vi "Dashboard Main.vi"() -> ()   [LabVIEW 2017]
uses:
  <vilib>/Rock Robotics/Network Tables/NT Read Numeric Array.vi
  <vilib>/Rock Robotics/Network Tables/NT Read Boolean.vi
  <vilib>/Rock Robotics/Network Tables/NT Read String.vi
  <vilib>/Rock Robotics/Network Tables/NT Read Number.vi
  <vilib>/Rock Robotics/WPI/Dashboard/WPI_DashboardLogging Global.vi
  <vilib>/Rock Robotics/Network Tables/NT Write Boolean.vi
  <vilib>/Rock Robotics/Network Tables/NT Read String Array.vi
  <vilib>/Rock Robotics/Network Tables/NT Write Number.vi
panel:
  in  "Camera Name":string(combo)="No Camera Selection"
  in  "Camera Settings Right":T1={"Frame Rate"=30, "Compression"=30, "Size"=1, "DB Camera Config"=FALSE} {"Frame Rate" scale=1.0..30.0; "Compression" scale=100.0..-1.0; "Size" items=["640x480", "320x240", "160x120"]}
  in  "Camera Name Right":string(combo)="No Camera Selection"
  out "Camera Info":cluster{"Mbps LED":bool, "Mbps":dbl, "fps":dbl} {"fps" format="%#.1g"; "Mbps" format="%#.1g"}
  in  "Camera Settings":T1={"Frame Rate"=30, "Compression"=30, "Size"=1, "DB Camera Config"=FALSE} {"Frame Rate" scale=1.0..30.0; "Compression" scale=100.0..-1.0; "Size" items=["640x480", "320x240", "160x120"]}
  in  "TCP":refnum<k5>
  in  "Rec Mode":enum32{"Stop", "Record", "Playback"}(radio)
  out "Robot IP":string
  out "Image Message":string="Timeout in Camera Communications"
  in  "Dashboard Tab":T2(tab)
  out "NT Connection":bool
  out "MotorChart R":cluster{"Numeric":dbl, "Numeric":dbl}(graph)
  out "MotorChart L":cluster{"Numeric":dbl, "Numeric":dbl}(graph)
  out "MotorSliders R":cluster{"MotorSlide1":dbl, "MotorSlide2":dbl} {"MotorSlide2" scale=-1.0..1.0 scale format="%#_2e"; "MotorSlide1" scale=-1.0..1.0 scale format="%#_2e"}
  out "MotorSliders L":cluster{"MotorSlide1":dbl, "MotorSlide2":dbl} {"MotorSlide2" scale=-1.0..1.0 scale format="%#_2e"; "MotorSlide1" scale=-1.0..1.0 scale format="%#_2e"}
  out "Gyro":dbl(knob) scale=0.0..360.0
  out "JS1 Z":dbl(slide) scale=-1.0..1.0 scale format="%#_2e"
  out "JS1 Graph":cluster{"X":dbl, "Y":dbl}[](graph)
  out "JS1 Buttons":T3
  out "JS2 Z":dbl(slide) scale=-1.0..1.0 scale format="%#_2e"
  out "JS2 Graph":cluster{"X":dbl, "Y":dbl}[](graph)
  out "JS2 Buttons":T3
  out "Mode":T4(ring)=enum."Auto Disabled"
  in  "Reload Auto Routines":bool
  in  "Starting Position":u16(ring) items=["Any", "Left", "Center", "Right"]
  in  "Run Auto In Teleop":bool
  in  "Right-Right-Right Routine":u16(ring) items=["Auto Line", "Auto Line (Reverse)", "Left Switch->Left Scale", "Left Switch->Left Switch->Left Scale", "Left Switch->Left Switch", "Left Switch->Left Switch (Back)", "Left Switch->Right Scale", "Left Switch", "Right Switch->Left Scale", "Right Switch->Right Scale", "Right Switch->Right Switch->Right Scale", "Right Switch->Right Switch", "Right Switch->Right Switch (Back)", "Right Switch"]
  in  "Right-Left-Right Routine":u16(ring) items=["Auto Line", "Auto Line (Reverse)", "Left Switch->Left Scale", "Left Switch->Left Switch->Left Scale", "Left Switch->Left Switch", "Left Switch->Left Switch (Back)", "Left Switch->Right Scale", "Left Switch", "Right Switch->Left Scale", "Right Switch->Right Scale", "Right Switch->Right Switch->Right Scale", "Right Switch->Right Switch", "Right Switch->Right Switch (Back)", "Right Switch"]
  in  "Left-Right-Left Routine":u16(ring) items=["Auto Line", "Auto Line (Reverse)", "Left Switch->Left Scale", "Left Switch->Left Switch->Left Scale", "Left Switch->Left Switch", "Left Switch->Left Switch (Back)", "Left Switch->Right Scale", "Left Switch", "Right Switch->Left Scale", "Right Switch->Right Scale", "Right Switch->Right Switch->Right Scale", "Right Switch->Right Switch", "Right Switch->Right Switch (Back)", "Right Switch"]
  in  "Left-Left-Left Routine":u16(ring) items=["Auto Line", "Auto Line (Reverse)", "Left Switch->Left Scale", "Left Switch->Left Switch->Left Scale", "Left Switch->Left Switch", "Left Switch->Left Switch (Back)", "Left Switch->Right Scale", "Left Switch", "Right Switch->Left Scale", "Right Switch->Right Scale", "Right Switch->Right Switch->Right Scale", "Right Switch->Right Switch", "Right Switch->Right Switch (Back)", "Right Switch"]
  out "RRR":string
  out "RLR":string
  out "LRL":string
  out "LLL":string
  out "Arm Control State":string
  out "Auto Control Active":bool
  out "Active Auto Routine":string
  out "Active Start Position":string
  out "Arm Rotate Limit Active":bool
  out "Arm Extend Limit Active":bool
  out "Arm Home Failure":bool
  out "Arm Home Success":bool
  out "Arm":cluster{dbl[], dbl[]}[](graph)
  out "Right Drive Zero":i32
  out "Left Drive Zero":i32
  in  "Reset Encoder Values":bool
  out "Right Drive":i32
  out "Left Drive":i32
  out "Tree":string(tree)
  out "Camera Image":T5(plugin-control)
  # "HW"
  # "HW"
  # "Joysticks"
  # "Drive Motors"
  # "Front"
  # "Right"
  # "Left"
  # "Back"
  # "Left Start"
  # "Center Start"
  # "Right Start"
  # "Armed Auto Routines"
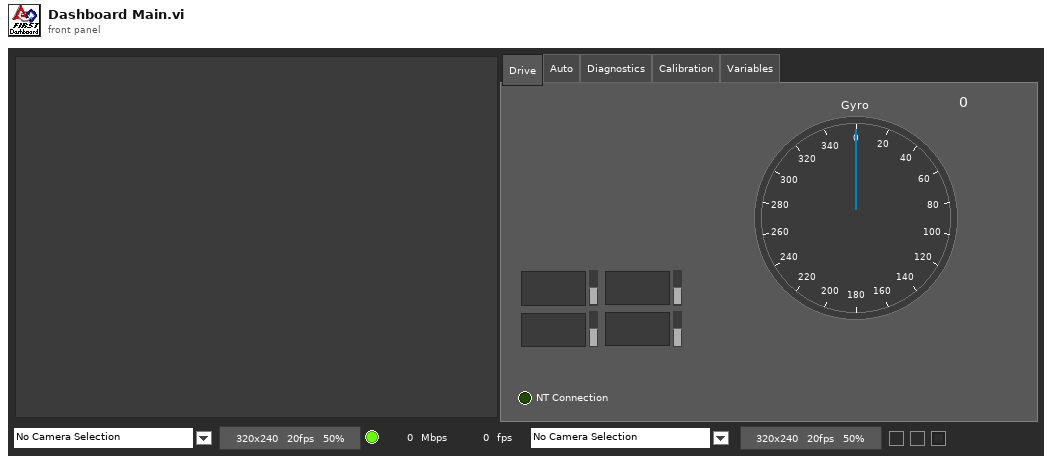
[diagram p1: front panel]
types:
  T1 = cluster{"Frame Rate":i32, "Compression":i32, "Size":u16, "DB Camera Config":bool}
  T2 = enum32{"Drive", "Auto", "Diagnostics", "Calibration", "Variables"}
  T3 = cluster{bool, bool, bool, bool, bool, bool, bool, bool, bool, bool, bool, bool}
  T4 = enum8{"Tele-Op Disabled", "Tele-Op Enabled", "Auto Disabled", "Auto Enabled", "Test Disabled", "Test Enabled", "Disconnected", "No Code", "E-Stop"}
  T5 = typedef "IMAQ Image.ctl" = refnum<image>
  T6 = enum32{"Drive", "Auto", "Diagnostics", "Variables"}
  T7 = cluster{"Save Path":path, "Interval (s)":dbl, "Keep":i32}
  T8 = typedef "Image Type" = u32
  T9 = cluster{"IDs":cluster{"RPC field ID":u16, "Unique ID":u16}, "String":string}
  T10 = cluster{"Error Strings":string, "Disable Counts":cluster{u16, u16}, "Rail Faults":cluster{u16, u16, u16}, "Robot IP":string, "DB Mode":u8, "Event Info":cluster{"Name":string, "Type":u8, "Number":u16, "Replay":u8}}
  T11 = cluster{"Storage":cluster{"Disk Free":u64, "RAM Block":u32, "RAM free":u32}, "CPU Utilization":cluster{"CPU % ISR":sgl, "CPU % Time Crit":sgl, "CPU % Timed Str":sgl, "CPU % High":sgl, "CPU % Above":sgl, "CPU % Normal":sgl, "CPU % Low":sgl}, "CAN":cluster{"% Bus Utilization":sgl, "Bus Off Cnt":u32, "TX_FIFO Full Cnt":u32, "Receive Error Cnt":u8, "Transmit Error Cnt":u8}, "HID":cluster{"HID Outputs":u32, "Rumble Low":u16, "Rumble High":u16}[]}
  T12 = cluster{"Status bits":cluster{"Test Mode":bool, "Autonomous":bool, "Enabled":bool, "Code Start":bool, "Brownout":bool, "Reserved 2":bool, "Reserved 3":bool, "E-Stop":bool}, "Code Trace":cluster{"Disabled":bool, "TeleOp":bool, "Auto":bool, "Test":bool}, "Controller Type":enum16{"unknown", "cRIO", "roboRio"}, "Code?":enum16{"unknown", "noCode", "code"}, "Battery V":dbl}
  T13 = cluster{"Control Bits":cluster{"TestMode":bool, "Autonomous":bool, "Enabled":bool, "FMS Present":bool, bool, bool, bool, "E-Stop":bool}, "Team Station ":u8, "Countdown":sgl, "Joystick Values":cluster{"Axes":dbl[], "Buttons":bool[], "POVs":i16[]}[]}
  T14 = cluster{"Axes":dbl[], "Buttons":bool[], "POVs":i16[]}[]
  T15 = cluster{"Axes":dbl[], "Buttons":bool[], "POVs":i16[]}
  T16 = cluster{"Buttons[0]":bool, "Buttons[1]":bool, "Buttons[2]":bool, "Buttons[3]":bool, "Buttons[4]":bool, "Buttons[5]":bool, "Buttons[6]":bool, "Buttons[7]":bool, "Buttons[8]":bool, "Buttons[9]":bool, "Buttons[10]":bool, "Buttons[11]":bool}
  T17 = cluster{"Camera Image":refnum<vi>, "Dashboard Tab":refnum<vi>, "Rec Mode":refnum<vi>, "Tree":refnum<vi>, "Camera Settings":refnum<vi>, "Camera Name":refnum<vi>, "Camera Info":refnum<vi>, "Camera Settings Right":refnum<vi>, "Camera Name Right":refnum<vi>}
  T18 = cluster{"Camera Name Right":string, string, "Saved DB Images Info":cluster{"Save Path":path, "Interval (s)":dbl, "Keep":i32}}
  T19 = cluster{"Camera Name":string, string, "Saved DB Images Info":cluster{"Save Path":path, "Interval (s)":dbl, "Keep":i32}}
  T20 = cluster{"Operation":enum16{"Update", "Clear"}, "Color Box":u32}[]
  T21 = cluster{"Image Size":bool, "Image Type":bool, "Pixel Value":bool, "ROI Information":bool, "Zoom Factor":bool}
  T22 = cluster{"Shift":bool, "Ctrl":bool, "Alt":bool, "Cmd":bool, "Opt":bool}
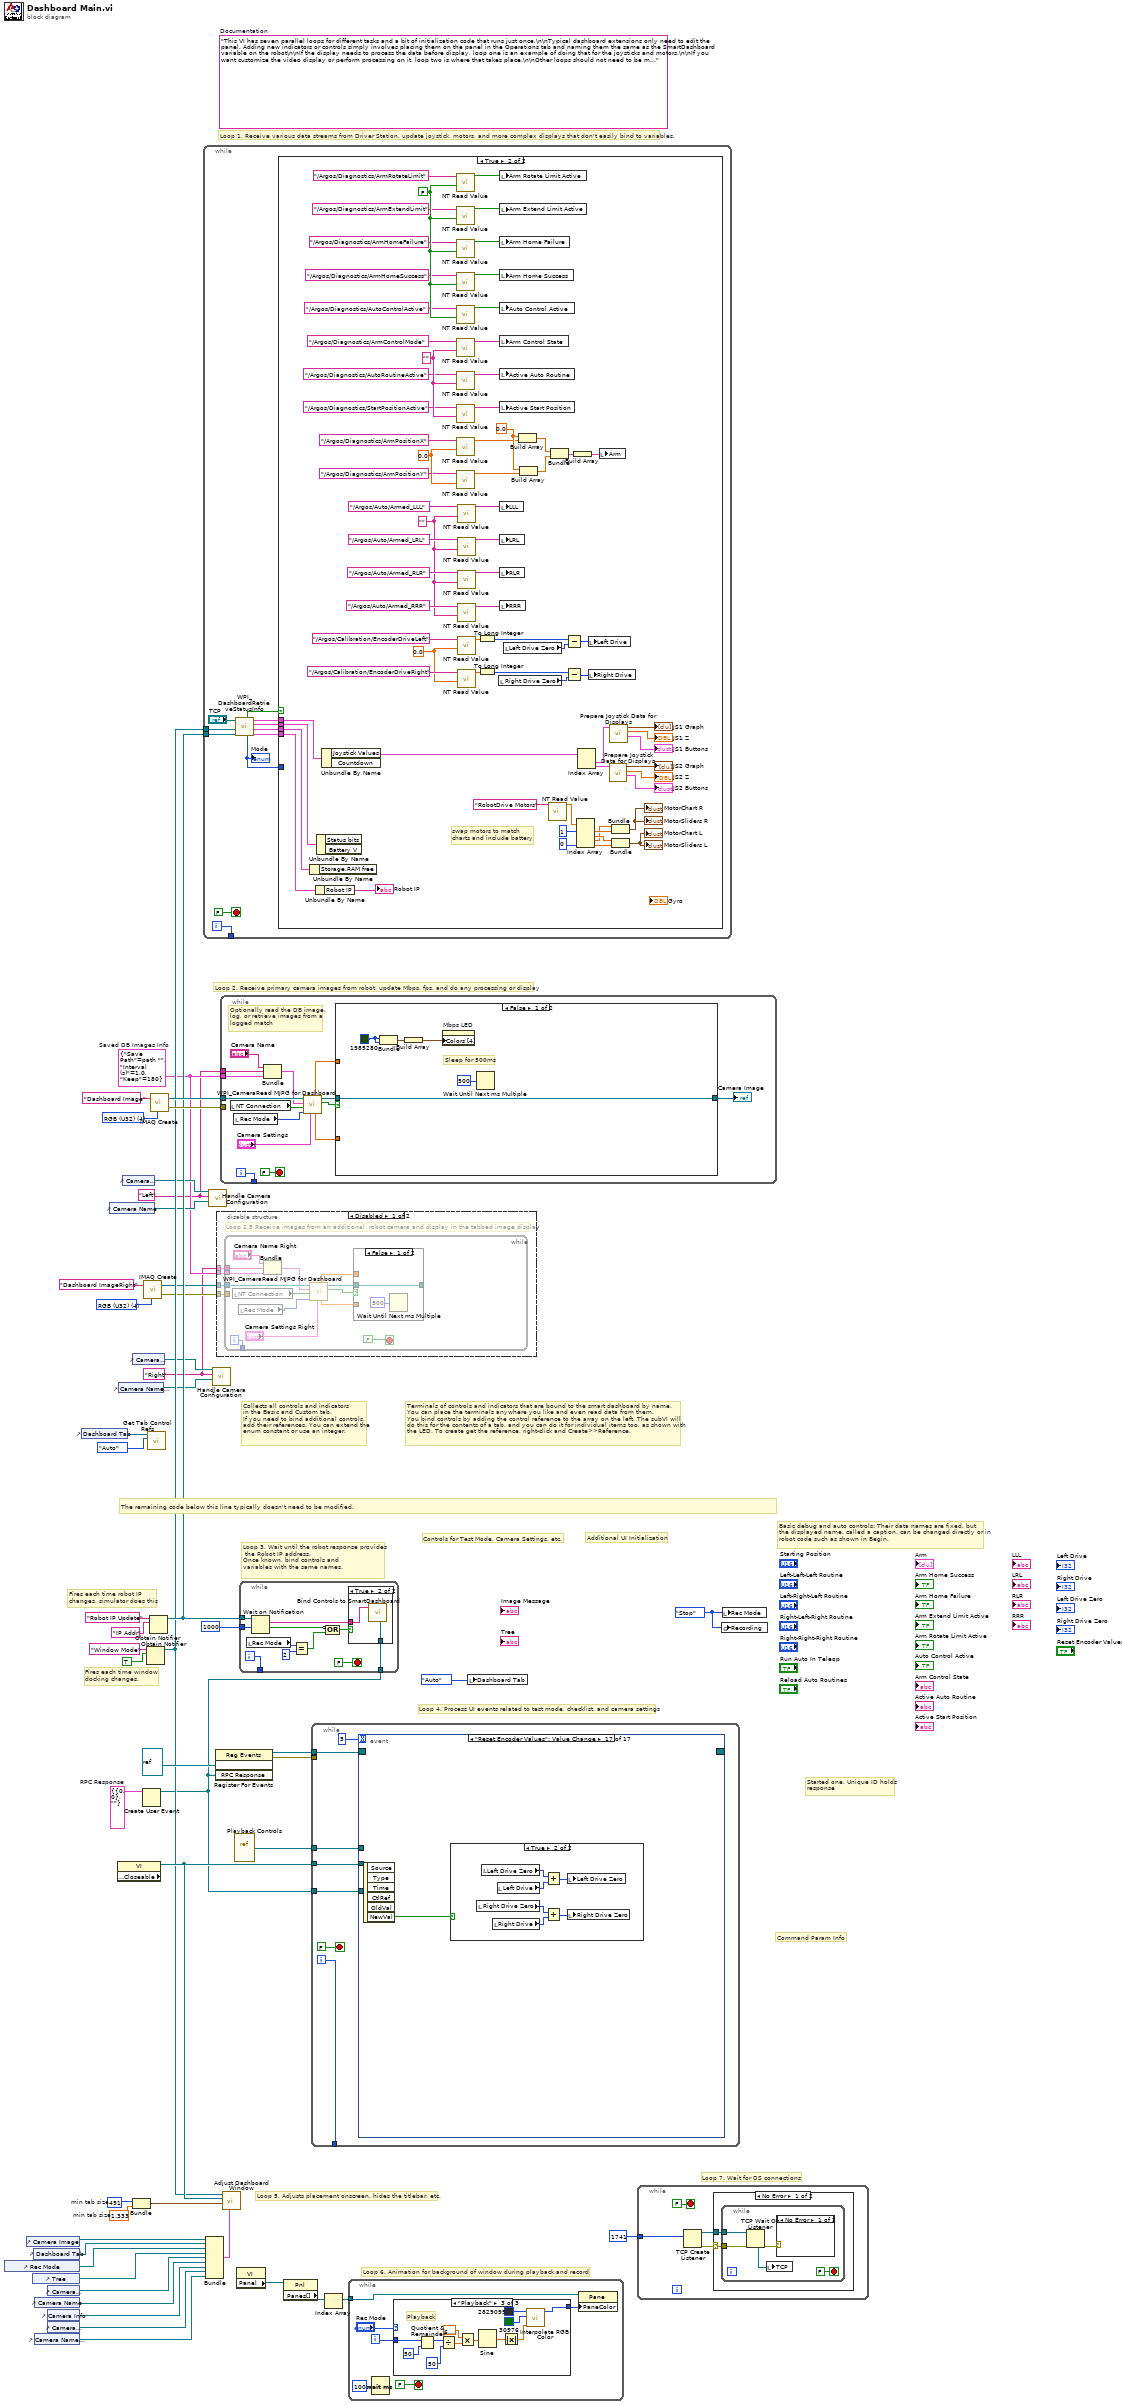
[diagram p0: block diagram]
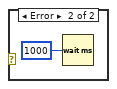
[diagram p5: hidden frame]
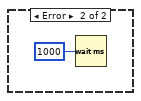
[diagram p6: hidden frame]
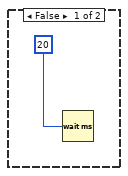
[diagram p7: hidden frame]
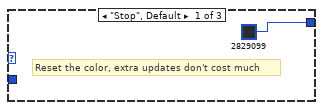
[diagram p8: hidden frame]
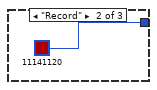
[diagram p9: hidden frame]
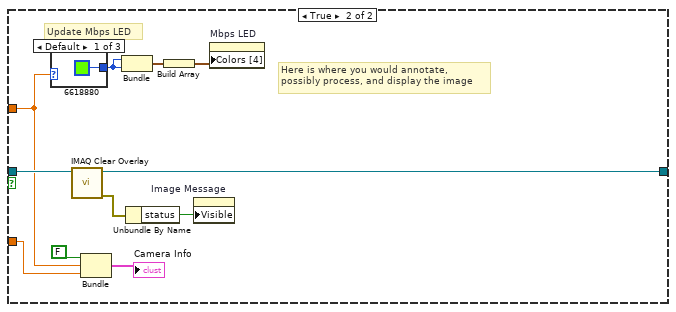
[diagram p10: hidden frame]
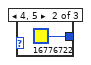
[diagram p11: hidden frame]
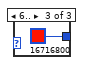
[diagram p12: hidden frame]
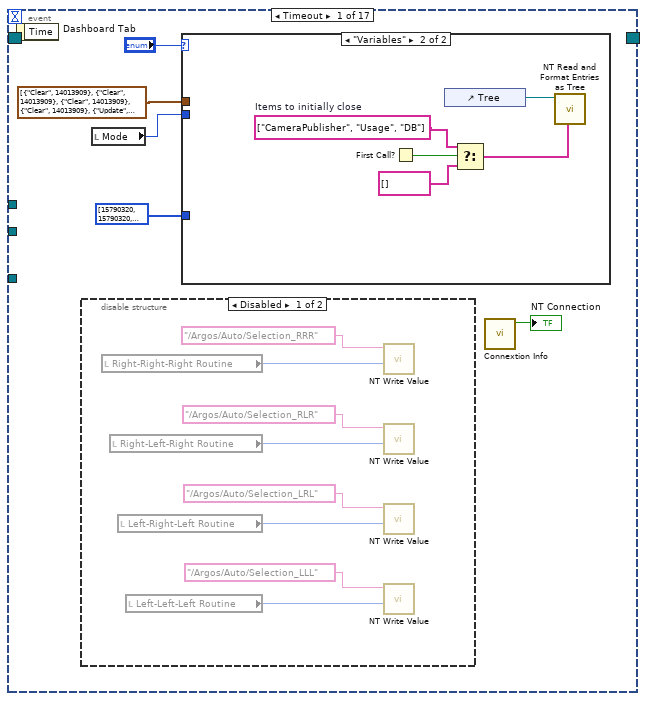
[diagram p13: hidden frame]
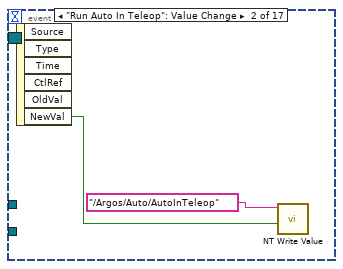
[diagram p16: hidden frame]
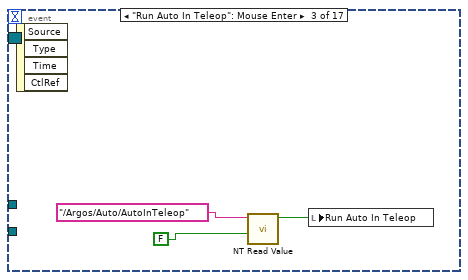
[diagram p17: hidden frame]
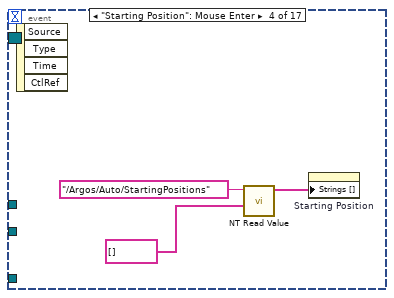
[diagram p18: hidden frame]
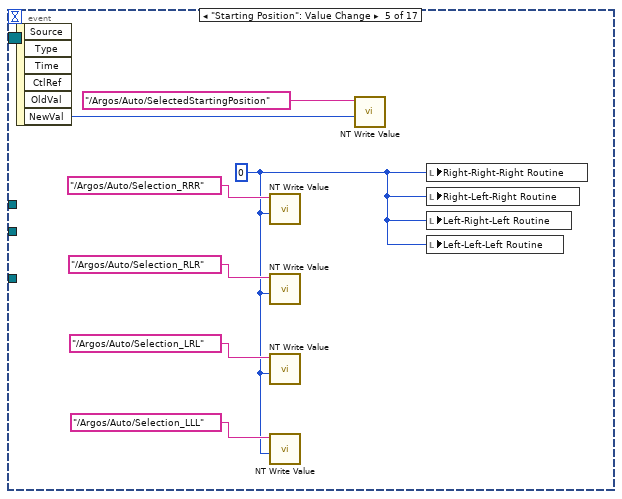
[diagram p19: hidden frame]
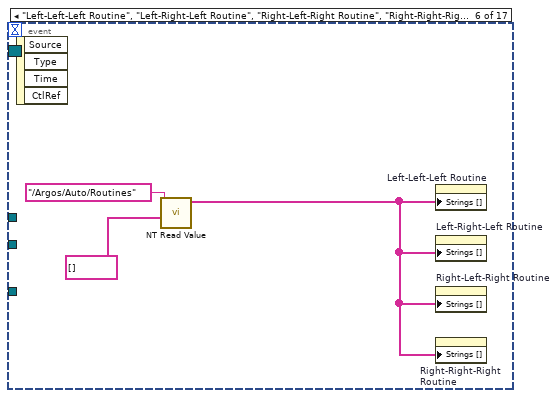
[diagram p20: hidden frame]
diagram:
  w5 = T7 {"Save Path"=path "", "Interval (s)"=1.0, "Keep"=180}  # Saved DB Images Info
  w4 = "Right"
  w3 = "Left"
  w12 = T8 4 items=["Grayscale (U8)", "Grayscale (I16)", "Grayscale (SGL)", "Complex (CSG)", "RGB (U32)", "HSL (U32)", "RGB (U64)"] ("Image Type")
  w20 = T9 {"IDs"={"RPC field ID"=0, "Unique ID"=0}, "String"=""}  # RPC Response
  w30 = 491  # min tab size
  w29 = 1.333  # min tab size
  w35 = enum32{"Stop", "Record", "Playback"}."Stop" ("Rec Mode")
  (unwired) "This VI has seven parallel loops for different tasks and a bit of initialization code that runs just once.\n\nTypical dashboard extensions only need to edit the panel. Adding new indicators or controls simply involves placing them on the panel in the Operations tab and naming them the same as the SmartDashboard variable on the robot\n\nIf the display needs to process the data before display, loop one is an example of doing that for the joysticks and motors.\n\nIf you want customize the video display or perform processing on it, loop two is where that takes place.\n\nOther loops should not need to be modified. They are pretty standard, and document the task they perform."  # Documentation
  w50 = T8 4 items=["Grayscale (U8)", "Grayscale (I16)", "Grayscale (SGL)", "Complex (CSG)", "RGB (U32)", "HSL (U32)", "RGB (U64)"] ("Image Type")
  # "Loop 3. Wait until the robot response provides\n the Robot IP address.\nOnce known, bind controls and\nvariables with the same names."
  # "Command Param Info"
  # "Started one, Unique ID holds\nresponse"
  # "Loop 7. Wait for DS connections"
  # "Basic debug and auto controls: Their data names are fixed, but\nthe displayed name, called a caption, can be changed directly or in\nrobot code such as shown in Begin."
  # "Controls for Test Mode, Camera Settings, etc."
  # "Additional UI Initialization"
  # "Loop 6. Animation for background of window during playback and record"
  # "Fires each time robot IP\nchanges, simulator does this"
  # "Fires each time window\ndocking changes."
  # "Collects all controls and indicators\nin the Basic and Custom tab.\nIf you need to bind additional controls,\nadd their references. You can extend the\nenum constant or use an integer."
  # "The remaining code below this line typically doesn't need to be modified."
  # "Loop 4. Process UI events related to test mode, checklist, and camera settings"
  # "Terminals of controls and indicators that are bound to the smart dashboard by name.\nYou can place the terminals anywhere you like and even read data from them.\nYou bind controls by adding the control reference to the array on the left. The subVI will\ndo this for the contents of a tab, and you can do it for individual items too, as shown with\nthe LED. To create get the reference, right-click and Create>>Reference."
  # "Loop 5. Adjusts placement onscreen, hides the titlebar, etc."
  # "Loop 1. Receive various data streams from Driver Station, update joystick, motors, and more complex displays that don't easily bind to variables."
  # "Loop 2. Receive primary camera images from robot, update Mbps, fps, and do any processing or display"
  n1 = control-ref of="Rec Mode"() -> (w25:refnum<vi>)
  n2 = control-ref of="Camera Image"() -> (w32:refnum<vi>)
  n3 = control-ref of="Tree"() -> (w26:refnum<vi>)
  n4 = control-ref of="Dashboard Tab"() -> (w31:refnum<vi>)
  n5 = control-ref of="Camera Name"() -> (w15:refnum<vi>)
  n6 = control-ref of="Camera Name Right"() -> (w6:refnum<vi>)
  n7 = control-ref of="Camera Settings"() -> (w16:refnum<vi>)
  n8 = control-ref of="Camera Info"() -> (w14:refnum<vi>)
  n9 = control-ref of="Camera Settings Right"() -> (w7:refnum<vi>)
  n10 = control-ref of="Dashboard Tab"() -> (w33:refnum<vi>)
  n11 = control-ref of="Camera Name"() -> (w17:refnum<vi>)
  n12 = property class="VI" props=["Front Panel.Closeable"]() -> (reference out=w34:refnum<vi>)  [unwired: 2 in, 2 out]
  n13 = control-ref of="Camera Name Right"() -> (w8:refnum<vi>)
  n14 = control-ref of="Camera Settings"() -> (w18:refnum<vi>)
  n15 = control-ref of="Camera Settings Right"() -> (w9:refnum<vi>)
  n16 = Bundle("min tab size"=w30, "min tab size"=w29) -> (w28:cluster{"min tab size":i32, "min tab size":dbl})  [unwired: 1 in]
  n17 = Create User Event(user event datatype=w20) -> (user event=w19:refnum<user-event>)  [unwired: 1 in, 1 out]
  n18 = call "IMAQ Create"("Image Name"="Dashboard ImageRight", "Image Type"=w12) -> ("New Image"=w11:T5, "error out"=w10:errorcluster)  [unwired: 2 in, 1 out]
  n19 = Obtain Notifier(name (unnamed)="Window Mode", notification data type=TRUE) -> (notifier out=w23:refnum<notifier>)  [unwired: 2 in, 2 out]
  n20 = call <vilib>:"Get Tab Control Refs.vi"("Page Index"=T6."Auto" ("Dashboard Tab"), "TabControl in"=w33) -> ()  [unwired: 9 in, 1 out]
  n21 = Obtain Notifier(name (unnamed)="Robot IP Update", notification data type="IP Addr" ("name (unnamed)")) -> (notifier out=w24:refnum<notifier>)  [unwired: 2 in, 2 out]
  n22 = call "IMAQ Create"("Image Name"="Dashboard Image", "Image Type"=w50) -> ("New Image"=w48:T5, "error out"=w47:errorcluster)  [unwired: 2 in, 1 out]
  n23 = while {
    tunnel: [w60] -> _
    tunnel: w24 -> [w54]
    tunnel: w23 -> [w51]
    i -> [w60]
    stop <- FALSE stop-if-true
    n24 = call <vilib>:"WPI_DashboardRetrieveStatusInfo.vi"("Binding Refnum"=w54, "Window Mode Notifier"=w51, "TCP Cnx"="TCP") -> ("Power and Errors"=w55:T10, "Robot Metrics"=w58:T11, "Status Info"=w59:T12, "Control Info"=w56:T13, "Robot Mode"=w53:T4, "Process?"=w57:bool)  [unwired: 3 in]
    "Mode" <- w53
    n25 = case shown="True" w57 {
      tunnel: w59 -> [_ w134]
      tunnel: w58 -> [_ w133]
      tunnel: w56 -> [_ w132]
      tunnel: w55 -> [_ w131]
      tunnel: w53 -> [_ _]
      frame False {
        n26 = Wait (ms)(milliseconds to wait=u32 20) -> ()  [unwired: 1 out]
      }
      frame True {
        w71 = 0.0 ("Default Value")
        w78 = "" ("Default Value")
        w88 = 0.0 ("Default Value")
        w93 = 0.0 ("element")
        w99 = "" ("Default Value")
        w110 = FALSE ("Default Value")
        # "swap motors to match\ncharts and include battery"
        n27 = Unbundle By Name(w133) -> ()  [unwired: 1 out]
        n28 = Unbundle By Name(w131) -> ("Robot IP"=→"Robot IP":string)
        n29 = Unbundle By Name(w134) -> ()  [unwired: 2 out]
        n30 = Unbundle By Name(w132) -> ("Joystick Values"=w122:T14)  [unwired: 1 out]
        n31 = call-poly <vilib>:"NT Read Value.vi"("Default Value"=w110, "Name"="/Argos/Diagnostics/ArmRotateLimit") -> ("Boolean"=w109:bool)  [unwired: 8 in, 1 out]
        n32 = call-poly <vilib>:"NT Read Value.vi"("Default Value"=w110, "Name"="/Argos/Diagnostics/ArmExtendLimit") -> ("Boolean"=w108:bool)  [unwired: 8 in, 1 out]
        n33 = call-poly <vilib>:"NT Read Value.vi"("Default Value"=w110, "Name"="/Argos/Diagnostics/ArmHomeFailure") -> ("Boolean"=w107:bool)  [unwired: 8 in, 1 out]
        n34 = call-poly <vilib>:"NT Read Value.vi"("Default Value"=w110, "Name"="/Argos/Diagnostics/ArmHomeSuccess") -> ("Boolean"=w106:bool)  [unwired: 8 in, 1 out]
        n35 = call-poly <vilib>:"NT Read Value.vi"("Default Value"=w110, "Name"="/Argos/Diagnostics/AutoControlActive") -> ("Boolean"=w105:bool)  [unwired: 8 in, 1 out]
        n36 = call-poly <vilib>:"NT Read Value.vi"("Default Value"=w99, "Name"="/Argos/Diagnostics/ArmControlMode") -> ("String"=w98:string)  [unwired: 8 in, 1 out]
        n37 = call-poly <vilib>:"NT Read Value.vi"("Default Value"=w99, "Name"="/Argos/Diagnostics/AutoRoutineActive") -> ("String"=w97:string)  [unwired: 8 in, 1 out]
        n38 = call-poly <vilib>:"NT Read Value.vi"("Default Value"=w99, "Name"="/Argos/Diagnostics/StartPositionActive") -> ("String"=w96:string)  [unwired: 8 in, 1 out]
        n39 = call-poly <vilib>:"NT Read Value.vi"("Default Value"=w88, "Name"="/Argos/Diagnostics/ArmPositionX") -> ("Numeric"=w92:dbl)  [unwired: 8 in, 1 out]
        n40 = call-poly <vilib>:"NT Read Value.vi"("Default Value"=w88, "Name"="/Argos/Diagnostics/ArmPositionY") -> ("Numeric"=w91:dbl)  [unwired: 8 in, 1 out]
        n41 = call-poly <vilib>:"NT Read Value.vi"("Default Value"=w78, "Name"="/Argos/Auto/Armed_LLL") -> ("String"=w77:string)  [unwired: 8 in, 1 out]
        n42 = call-poly <vilib>:"NT Read Value.vi"("Default Value"=w78, "Name"="/Argos/Auto/Armed_LRL") -> ("String"=w76:string)  [unwired: 8 in, 1 out]
        n43 = call-poly <vilib>:"NT Read Value.vi"("Default Value"=w78, "Name"="/Argos/Auto/Armed_RLR") -> ("String"=w75:string)  [unwired: 8 in, 1 out]
        n44 = call-poly <vilib>:"NT Read Value.vi"("Default Value"=w78, "Name"="/Argos/Auto/Armed_RRR") -> ("String"=w74:string)  [unwired: 8 in, 1 out]
        n45 = call-poly <vilib>:"NT Read Value.vi"("Default Value"=w71, "Name"="/Argos/Calibration/EncoderDriveLeft") -> ("Numeric"=w70:dbl)  [unwired: 8 in, 1 out]
        n46 = call-poly <vilib>:"NT Read Value.vi"("Default Value"=w71, "Name"="/Argos/Calibration/EncoderDriveRight") -> ("Numeric"=w69:dbl)  [unwired: 8 in, 1 out]
        n47 = To Long Integer(number=w70) -> (32bit integer=w64:i32)
        n48 = To Long Integer(number=w69) -> (32bit integer=w67:i32)
        n49 = local read "Right Drive Zero"() -> (w66:i32)
        n50 = local write "Arm Rotate Limit Active"(w109) -> ()
        n51 = local write "Arm Extend Limit Active"(w108) -> ()
        n52 = local write "Arm Home Failure"(w107) -> ()
        n53 = local write "Arm Home Success"(w106) -> ()
        n54 = local write "Auto Control Active"(w105) -> ()
        n55 = local write "Arm Control State"(w98) -> ()
        n56 = local write "Active Auto Routine"(w97) -> ()
        n57 = local write "Active Start Position"(w96) -> ()
        n58 = local write "LLL"(w77) -> ()
        n59 = local write "LRL"(w76) -> ()
        n60 = local write "RLR"(w75) -> ()
        n61 = local write "RRR"(w74) -> ()
        n62 = local read "Left Drive Zero"() -> (w63:i32)
        n63 = Build Array(w93, w92) -> (w95:dbl[])
        n64 = Build Array(w93, w91) -> (w94:dbl[])
        n65 = call-poly <vilib>:"NT Read Value.vi"("Name"="RobotDrive Motors") -> ("Numeric Array"=w112:dbl[])  [unwired: 9 in, 1 out]
        n66 = Bundle(w95, w94) -> (w90:cluster{dbl[], dbl[]})  [unwired: 1 in]
        n67 = Subtract(x=w64, y=w63) -> (x-y=w65:i32)
        n68 = Subtract(x=w67, y=w66) -> (x-y=w68:i32)
        n69 = Build Array(w90) -> (w89:cluster{dbl[], dbl[]}[])
        n70 = Index Array(array=w112, index #1=1, index #4=0) -> (element #1=w126:dbl, element #2=w127:dbl, element #3=w125:dbl, element #4=w130:dbl)  [unwired: 2 in]
        n71 = Index Array(array=w122) -> (element #1=w121:T15, element #2=w117:T15)  [unwired: 2 in]
        n72 = local write "Left Drive"(w65) -> ()
        n73 = local write "Right Drive"(w68) -> ()
        n74 = local write "Arm"(w89) -> ()
        n75 = call "Prepare Joystick Data for Displays.vi"("Joystick Values"=w117) -> ("Buttons"=→"JS2 Buttons":T16, "Z Axis"=→"JS2 Z":dbl, "Cartesian Data"=→"JS2 Graph":cluster{"X axis":dbl, "X axis":dbl}[])  [unwired: 8 in]
        n76 = call "Prepare Joystick Data for Displays.vi"("Joystick Values"=w121) -> ("Buttons"=→"JS1 Buttons":T16, "Z Axis"=→"JS1 Z":dbl, "Cartesian Data"=→"JS1 Graph":cluster{"X axis":dbl, "X axis":dbl}[])  [unwired: 8 in]
        n77 = Bundle("Numeric"=w125, "Numeric"=w126) -> (→"MotorChart R" →"MotorSliders R":cluster{"Numeric":dbl, "Numeric":dbl})  [unwired: 1 in]
        n78 = Bundle("Numeric"=w127, "Numeric"=w130) -> (→"MotorChart L" →"MotorSliders L":cluster{"Numeric":dbl, "Numeric":dbl})  [unwired: 1 in]
      }
    }
  }
  n79 = Bundle("Camera Image"=w32, "Dashboard Tab"=w31, "Rec Mode"=w25, "Tree"=w26, "Camera Settings"=w16, "Camera Name"=w15, "Camera Info"=w14, "Camera Settings Right"=w7, "Camera Name Right"=w6) -> (w27:T17)  [unwired: 1 in]
  n80 = call "Handle Camera Configuration.vi"("CameraNameRef"=w17, "Display Name"=w3, "ClusterRef"=w18) -> ()  [unwired: 9 in]
  n81 = call "Handle Camera Configuration.vi"("CameraNameRef"=w8, "Display Name"=w4, "ClusterRef"=w9) -> ()  [unwired: 9 in]
  n82 = register-events(refnum<vi> refnum, w19) -> (reference out=w38:refnum<event-registration>, error out=w37:errorcluster)  [unwired: 2 in]
  n83 = disable-structure shown="Disabled" {
    disable-tunnel: w11 -> [w138 _]
    disable-tunnel: w10 -> [w137 _]
    disable-tunnel: w5 -> [w136 _]
    disable-tunnel: w4 -> [w135 _]
    frame Disabled {
      # "Loop 2.5 Receive images from an additional  robot camera and display in the tabbed image display"
      n84 = while {
        tunnel: w138 -> [w152]
        tunnel: w137 -> [_]
        tunnel: [w147] -> _
        tunnel: w136 -> [w142]
        tunnel: w135 -> [w139]
        i -> [w147]
        stop <- FALSE stop-if-true
        n85 = local read "NT Connection"() -> (w143:bool)
        n86 = local read "Rec Mode"() -> (w151:enum32{"Stop", "Record", "Playback"})
        n87 = Bundle("Camera Name Right"="Camera Name Right", w139, "Saved DB Images Info"=w142) -> (w141:T18)  [unwired: 1 in]
        n88 = call <vilib>:"WPI_CameraRead MJPG for Dashboard.vi"("Camera Settings"="Camera Settings Right", "Rec Mode"=w151, "NT Connection"=w143, "Capture Info"=w141, "Refnum in"=w152) -> ("Active"=w146:bool, "Refnum out"=w149:T5, "FPS"=w144:dbl, "Bandwidth (Mbps)"=w145:dbl)  [unwired: 3 in]
        n89 = case shown="False" w146 {
          tunnel: w149 -> [w153 w155]
          tunnel: w145 -> [_ _]
          tunnel: w144 -> [_ _]
          tunnel: [w153 w155] -> _
          frame False {
            n90 = Wait Until Next ms Multiple(millisecond multiple=u32 500) -> ()  [unwired: 1 out]
          }
          frame True {
          }
        }
      }
    }
    frame Enabled {
    }
  }
  n91 = while {
    tunnel: w48 -> [w168]
    tunnel: w47 -> [_]
    tunnel: [w169] -> _
    tunnel: w5 -> [w159]
    tunnel: w3 -> [w156]
    i -> [w169]
    stop <- FALSE stop-if-true
    # "Optionally read the DB image,\nlog, or retrieve images from a\nlogged match"
    n92 = local read "NT Connection"() -> (w160:bool)
    n93 = local read "Rec Mode"() -> (w164:enum32{"Stop", "Record", "Playback"})
    n94 = Bundle("Camera Name"="Camera Name", w156, "Saved DB Images Info"=w159) -> (w158:T19)  [unwired: 1 in]
    n95 = call <vilib>:"WPI_CameraRead MJPG for Dashboard.vi"("Camera Settings"="Camera Settings", "Rec Mode"=w164, "NT Connection"=w160, "Capture Info"=w158, "Refnum in"=w168) -> ("Active"=w166:bool, "Refnum out"=w167:T5, "FPS"=w165:dbl, "Bandwidth (Mbps)"=w163:dbl)  [unwired: 3 in]
    n96 = case shown="False" w166 {
      tunnel: w167 -> [w171 w182]
      tunnel: w163 -> [_ w179]
      tunnel: w165 -> [_ w180]
      tunnel: [w171 w176] -> w161
      frame False {
        w173 = u32 1985280 ("Color Box")
        # "Sleep for 500ms"
        n97 = Bundle("Color Box"=w173, "Color Box"=w173) -> (w174:cluster{"Color Box":u32, "Color Box":u32})  [unwired: 1 out]
        n98 = Build Array(w174) -> (w172:cluster{"Color Box":u32, "Color Box":u32}[])
        n99 = property on="Mbps LED" class="Bool (strict)"("Colors [4]"=w172) -> ()  [unwired: 2 in, 2 out]
        n100 = Wait Until Next ms Multiple(millisecond multiple=u32 500) -> ()  [unwired: 1 out]
      }
      frame True {
        # "Here is where you would annotate,\npossibly process, and display the image"
        # "Update Mbps LED"
        n101 = case shown="Default" w179 {
          tunnel: [u32 6618880 ("Color Box") u32 16776722 ("Color Box") u32 16716800 ("Color Box")] -> w183
          frame Default {
          }
          frame 4, 5 {
          }
          frame 6.. {
          }
        }
        n102 = call "IMAQ Clear Overlay"("Image"=w182) -> ("error out"=w185:errorcluster, "Image Out"=w176:T5)  [unwired: 2 in, 7 out]
        n103 = Bundle(FALSE, "Bandwidth (Mbps)"=w179, "FPS"=w180) -> (→"Camera Info":cluster{bool, "Bandwidth (Mbps)":dbl, "FPS":dbl})  [unwired: 1 in]
        n104 = Bundle("Color Box"=w183, "Color Box"=w183) -> (w184:cluster{"Color Box":u32, "Color Box":u32})  [unwired: 1 out]
        n105 = Unbundle By Name(w185) -> ("status"=w186:bool)
        n106 = Build Array(w184) -> (w181:cluster{"Color Box":u32, "Color Box":u32}[])
        n107 = property on="Image Message" class="Str"("Visible"=w186) -> ()  [unwired: 2 in, 2 out]
        n108 = property on="Mbps LED" class="Bool (strict)"("Colors [4]"=w181) -> ()  [unwired: 2 in, 2 out]
      }
    }
    "Camera Image" <- w161
  }
  n109 = call "Adjust Dashboard Window.vi"("Sizing Refnums"=w27, "Size Constraints"=w28, "VI"=w34, "WIn Mode"=w23) -> ()  [unwired: 8 in]
  n110 = vi-ref "Playback Controls.vi"() -> (w39:refnum<vi>)
  n111 = property class="VI"() -> ("Panel"=w41:refnum<vi>)  [unwired: 2 in, 2 out]
  n112 = while {
    tunnel: w24 -> [w199]
    tunnel: [w197] -> _
    tunnel: u32 1000 ("milliseconds to wait") -> [w196]
    tunnel: w19 -> [w190]
    i -> [w197]
    stop <- FALSE stop-if-true
    n113 = local read "Rec Mode"() -> (w192:enum32{"Stop", "Record", "Playback"})
    n114 = Wait on Notification(notifier=w199, timeout in ms (-1)=w196) -> (notification=w198:string, timed out?=w194:bool)  [unwired: 2 in, 2 out]
    n115 = Equal?(x=w192, y=u16 2 ("Rec Mode")) -> (x = y?=w193:bool)
    n116 = Compound Arithmetic op=OR(invert w194, w193) -> (w195:bool)
    n117 = case shown="True" w195 {
      tunnel: w198 -> [_ w202]
      tunnel: w190 -> [_ w201]
      frame False {
      }
      frame True {
        n118 = call <vilib>:"Bind Controls to SmartDashboard.vi"("RPC ref"=w201, "Server IP Address"=w202) -> ()  [unwired: 10 in]
      }
    }
  }
  n119 = property class="Pnl"(reference=w41) -> ("Panes[]"=w42:refnum<vi>[])  [unwired: 1 in, 2 out]
  n120 = while {
    tunnel: [w207] -> _
    tunnel: w39 -> [w206]
    tunnel: w38 -> [w205]
    tunnel: w37 -> [_]
    tunnel: w34 -> [w204]
    tunnel: w19 -> [w203]
    i -> [w207]
    stop <- FALSE stop-if-true
    n121 = event shown="[16] \"Reset Encoder Values\": Value Change" {
      selector: w205 -> [_ _ _ _ _ _ _ _ _ _ _ _ _ _ _ _ _]
      dyn-events: [_ _ _ _ _ _ _ _ _ _ _ _ w265 _ _ _ _] -> _
      timeout: u32 5 ("milliseconds to wait") -> [_ _ _ _ _ _ _ _ _ _ _ _ _ _ _ _ _]
      tunnel: w206 -> [_ _ _ _ _ _ _ _ _ _ _ _ w267 _ w283 _ _]
      tunnel: w204 -> [_ _ _ _ _ _ _ _ _ _ _ _ w263 _ _ _ _]
      tunnel: w203 -> [_ _ _ _ _ _ _ _ _ _ _ _ w261 _ _ _ _]
      event Timeout {
        n122 = event-data() -> ()  [unwired: 1 in, 1 out]
        n123 = disable-structure shown="Disabled" {
          frame Disabled {
            n124 = local read "Right-Right-Right Routine"() -> (w219:u16)
            n125 = local read "Right-Left-Right Routine"() -> (w220:u16)
            n126 = local read "Left-Right-Left Routine"() -> (w222:u16)
            n127 = local read "Left-Left-Left Routine"() -> (w221:u16)
            n128 = call-poly <vilib>:"NT Write Value.vi"("Numeric"=w219, "Name"="/Argos/Auto/Selection_RRR") -> ()  [unwired: 9 in, 1 out]
            n129 = call-poly <vilib>:"NT Write Value.vi"("Numeric"=w220, "Name"="/Argos/Auto/Selection_RLR") -> ()  [unwired: 9 in, 1 out]
            n130 = call-poly <vilib>:"NT Write Value.vi"("Numeric"=w222, "Name"="/Argos/Auto/Selection_LRL") -> ()  [unwired: 9 in, 1 out]
            n131 = call-poly <vilib>:"NT Write Value.vi"("Numeric"=w221, "Name"="/Argos/Auto/Selection_LLL") -> ()  [unwired: 9 in, 1 out]
          }
          frame Enabled {
          }
        }
        n132 = local read "Mode"() -> (w211:T4)
        n133 = case shown="\"Variables\"" "Dashboard Tab" {
          tunnel: T20 [{"Operation"=enum."Clear", "Color Box"=14013909}, {"Operation"=enum."Clear", "Color Box"=14013909}, {"Operation"=enum."Clear", "Color Box"=14013909}, {"Operation"=enum."Clear", "Color Box"=14013909}, {"Operation"=enum."Update", "Color Box"=14013909}, {"Operation"=enum."Update", "Color Box"=16777215}, {"Operation"=enum."Clear", "Color Box"=14013909}, {"Operation"=enum."Clear", "Color Box"=14013909}, {"Operation"=enum."Clear", "Color Box"=14013909}] -> [_ _]
          tunnel: w211 -> [_ _]
          tunnel: u32[] [15790320, 15790320, 15790320, 15790320, 16777215, 16777215, 15790320, 15790320, 15790320] -> [_ _]
          frame "Diagnostics", Default {
          }
          frame "Variables" {
            w225 = string[] ["CameraPublisher", "Usage", "DB"]  # Items to initially close
            n134 = First Call?() -> (First Call?: T/F=w226:bool)
            n135 = control-ref of="Tree"() -> (w227:refnum<vi>)
            n136 = Select(t=w225, s=w226, f=string[] []) -> (s? t:f=w223:string[])
            n137 = call <vilib>:"NT Read and Format Entries as Tree.vi"("Tags to  Close"=w223, "Tree Refnum"=w227) -> ()  [unwired: 8 in, 2 out]
          }
        }
        n138 = call <vilib>:"Connextion Info.vi"() -> ("Connected"=→"NT Connection":bool)  [unwired: 10 in, 1 out]
      }
      event "Run Auto In Teleop": Value Change {
        n139 = event-data() -> ("NewVal"=w229:bool)  [unwired: 1 in, 5 out]
        n140 = call-poly <vilib>:"NT Write Value.vi"("Boolean"=w229, "Name"="/Argos/Auto/AutoInTeleop") -> ()  [unwired: 9 in, 1 out]
      }
      event "Run Auto In Teleop": Mouse Enter {
        n141 = event-data() -> ()  [unwired: 1 in, 4 out]
        n142 = call-poly <vilib>:"NT Read Value.vi"("Default Value"=FALSE, "Name"="/Argos/Auto/AutoInTeleop") -> ("Boolean"=w230:bool)  [unwired: 8 in, 1 out]
        n143 = local write "Run Auto In Teleop"(w230) -> ()
      }
      event "Starting Position": Mouse Enter {
        n144 = event-data() -> ()  [unwired: 1 in, 4 out]
        n145 = call-poly <vilib>:"NT Read Value.vi"("Default Value"=string[] [], "Name"="/Argos/Auto/StartingPositions") -> ("String Array"=w233:string[])  [unwired: 8 in, 1 out]
        n146 = property on="Starting Position" class="Ring (strict)"("Strings []"=w233) -> ()  [unwired: 2 in, 2 out]
      }
      event "Starting Position": Value Change {
        w236 = u16 0
        n147 = event-data() -> ("NewVal"=w241:u16)  [unwired: 1 in, 5 out]
        n148 = call-poly <vilib>:"NT Write Value.vi"("Numeric"=w236, "Name"="/Argos/Auto/Selection_RRR") -> ()  [unwired: 9 in, 1 out]
        n149 = call-poly <vilib>:"NT Write Value.vi"("Numeric"=w236, "Name"="/Argos/Auto/Selection_RLR") -> ()  [unwired: 9 in, 1 out]
        n150 = call-poly <vilib>:"NT Write Value.vi"("Numeric"=w236, "Name"="/Argos/Auto/Selection_LRL") -> ()  [unwired: 9 in, 1 out]
        n151 = call-poly <vilib>:"NT Write Value.vi"("Numeric"=w236, "Name"="/Argos/Auto/Selection_LLL") -> ()  [unwired: 9 in, 1 out]
        n152 = call-poly <vilib>:"NT Write Value.vi"("Numeric"=w241, "Name"="/Argos/Auto/SelectedStartingPosition") -> ()  [unwired: 9 in, 1 out]
        n153 = local write "Right-Right-Right Routine"(w236) -> ()
        n154 = local write "Right-Left-Right Routine"(w236) -> ()
        n155 = local write "Left-Right-Left Routine"(w236) -> ()
        n156 = local write "Left-Left-Left Routine"(w236) -> ()
      }
      event "Left-Left-Left Routine", "Left-Right-Left Routine", "Right-Left-Right Routine", "Right-Right-Right Routine": Mouse Enter {
        n157 = event-data() -> ()  [unwired: 1 in, 4 out]
        n158 = call-poly <vilib>:"NT Read Value.vi"("Default Value"=string[] [], "Name"="/Argos/Auto/Routines") -> ("String Array"=w243:string[])  [unwired: 8 in, 1 out]
        n159 = property on="Left-Left-Left Routine" class="Ring (strict)"("Strings []"=w243) -> ()  [unwired: 2 in, 2 out]
        n160 = property on="Left-Right-Left Routine" class="Ring (strict)"("Strings []"=w243) -> ()  [unwired: 2 in, 2 out]
        n161 = property on="Right-Left-Right Routine" class="Ring (strict)"("Strings []"=w243) -> ()  [unwired: 2 in, 2 out]
        n162 = property on="Right-Right-Right Routine" class="Ring (strict)"("Strings []"=w243) -> ()  [unwired: 2 in, 2 out]
      }
      event "Left-Left-Left Routine": Value Change {
        n163 = event-data() -> ()  [unwired: 1 in, 6 out]
        n164 = local read "Left-Left-Left Routine"() -> (w247:u16)
        n165 = call-poly <vilib>:"NT Write Value.vi"("Numeric"=w247, "Name"="/Argos/Auto/Selection_LLL") -> ()  [unwired: 9 in, 1 out]
      }
      event "Right-Right-Right Routine": Value Change {
        n166 = event-data() -> ()  [unwired: 1 in, 6 out]
        n167 = local read "Right-Right-Right Routine"() -> (w249:u16)
        n168 = call-poly <vilib>:"NT Write Value.vi"("Numeric"=w249, "Name"="/Argos/Auto/Selection_RRR") -> ()  [unwired: 9 in, 1 out]
      }
      event "Right-Left-Right Routine": Value Change {
        n169 = event-data() -> ()  [unwired: 1 in, 6 out]
        n170 = local read "Right-Left-Right Routine"() -> (w251:u16)
        n171 = call-poly <vilib>:"NT Write Value.vi"("Numeric"=w251, "Name"="/Argos/Auto/Selection_RLR") -> ()  [unwired: 9 in, 1 out]
      }
      event "Left-Right-Left Routine": Value Change {
        n172 = event-data() -> ()  [unwired: 1 in, 6 out]
        n173 = local read "Left-Right-Left Routine"() -> (w253:u16)
        n174 = call-poly <vilib>:"NT Write Value.vi"("Numeric"=w253, "Name"="/Argos/Auto/Selection_LRL") -> ()  [unwired: 9 in, 1 out]
      }
      event "Reload Auto Routines": Mouse Enter {
        n175 = event-data() -> ()  [unwired: 1 in, 4 out]
        n176 = call-poly <vilib>:"NT Read Value.vi"("Default Value"=FALSE, "Name"="/Argos/Auto/ReloadRoutines") -> ("Boolean"=w256:bool)  [unwired: 8 in, 1 out]
        n177 = local write "Reload Auto Routines"(w256) -> ()
      }
      event "Reload Auto Routines": Value Change {
        n178 = event-data() -> ("NewVal"=w257:bool)  [unwired: 1 in, 5 out]
        n179 = call-poly <vilib>:"NT Write Value.vi"("Boolean"=w257, "Name"="/Argos/Auto/ReloadRoutines") -> ()  [unwired: 9 in, 1 out]
      }
      event "Rec Mode": Value Change {
        # "Update globals for recording mode and path to read log from.\nClear when logging and let NetworkTables set path for vision to\nuse."
        n180 = event-data() -> ("NewVal"=w268:enum32{"Stop", "Record", "Playback"})  [unwired: 1 in]
        n181 = global write "WPI_DashboardLogging Global.vi" "Logging Filename"(path "") -> ()
        n182 = global write "WPI_DashboardLogging Global.vi" "Recording"(w268) -> ()
        n183 = case shown="\"Playback\"" w268 {
          tunnel: w267 -> [_ w270 w279]
          tunnel: [_ _ w278] -> w265
          tunnel: [_ _ w277] -> _
          tunnel: w263 -> [_ _ w275]
          tunnel: cluster{i32, i32} {-250, 170} -> [_ _ w274]
          tunnel: [_ _ T21 {"Image Size"=TRUE, "Image Type"=TRUE, "Pixel Value"=TRUE, "ROI Information"=TRUE, "Zoom Factor"=FALSE} ("Image Information Shown:All Elements")] -> w259
          tunnel: [_ _ TRUE ("Zoom Factor")] -> w260
          tunnel: w261 -> [_ _ w271]
          frame Default {
          }
          frame "Stop", "Record" {
            # "Place Window too"
            n184 = invoke class="VI" method="FP.Close"(reference=w270) -> (reference out=w269:refnum<vi>)  [unwired: 2 in, 2 out]
            n185 = invoke class="VI" method="Abort VI"(reference=w269) -> ()  [unwired: 2 in, 3 out]
          }
          frame "Playback" {
            n186 = call "Open Playback Panel.vi"("Offset"=w274, "DB VI Ref"=w275, "Playback in"=w279) -> ("Playback out"=w276:refnum<vi>)  [unwired: 8 in]
            n187 = register-events(w276, w271) -> (reference out=w278:refnum<event-registration>, error out=w277:errorcluster)  [unwired: 2 in]
          }
        }
        n188 = property on="Camera Image" class="ImageControl"("Image Information Shown"=w259, "Image Information Visible"=w260) -> ()  [unwired: 2 in, 2 out]
        n189 = call <vilib>:"WPI_DashboardNT Log FieldName Cache.vi"("Operation"=enum16{"Lookup/Add", "Index", "Clear"}."Clear") -> ()  [unwired: 8 in, 3 out]
      }
      event Panel Close {
        w280 = enum32{"Stop", "Record", "Playback"}."Stop" ("Rec Mode")
        # "Playback window has been closed, abort"
        n190 = event-data() -> ()  [unwired: 1 in, 4 out]
        n191 = local write "Rec Mode"(w280) -> ()
        n192 = global write "WPI_DashboardLogging Global.vi" "Recording"(w280) -> ()
      }
      event Panel Close {
        # "Abort playback window and ourself"
        n193 = event-data() -> ()  [unwired: 1 in, 4 out]
        n194 = invoke class="VI" method="FP.Close"(reference=w283) -> (reference out=w282:refnum<vi>)  [unwired: 2 in, 2 out]
        n195 = invoke class="VI" method="Abort VI"(reference=w282) -> (error out=w281:errorcluster)  [unwired: 2 in, 2 out]
        n196 = invoke class="VI" method="Abort VI"(error in=w281) -> ()  [unwired: 2 in, 3 out]
      }
      event "Tree": Double Click {
        n197 = event-data() -> ("PlatMods"=w289:T22, "Tag"=w286:string)  [unwired: 1 in]
        n198 = Unbundle(w289) -> ("Shift"=w288:bool)  [unwired: 4 out]
        n199 = String Subset(string=w286, length (rest)=1 ("length (rest)")) -> (substring=w285:string)  [unwired: 1 in]
        n200 = Not(x=w288) -> (.not. x?=w287:bool)
        n201 = case shown="\"/\"" w285 {
          tunnel: w286 -> [_ w291]
          tunnel: w287 -> [_ w290]
          frame Default {
          }
          frame "/" {
            n202 = call <vilib>:"NT Update Persistence.vi"("Persistence"=w290, "Name"=w291) -> ()  [unwired: 9 in, 1 out]
          }
        }
      }
      event "Reset Encoder Values": Value Change {
        n203 = event-data() -> ("NewVal"=w292:bool)  [unwired: 1 in, 5 out]
        n204 = case shown="True" w292 {
          frame False {
          }
          frame True {
            n205 = local read "Right Drive Zero"() -> (w298:i32)
            n206 = local read "Left Drive Zero"() -> (w295:i32)
            n207 = local read "Right Drive"() -> (w297:i32)
            n208 = local read "Left Drive"() -> (w294:i32)
            n209 = Add(x=w295, y=w294) -> (x+y=w293:i32)
            n210 = Add(x=w298, y=w297) -> (x+y=w296:i32)
            n211 = local write "Left Drive Zero"(w293) -> ()
            n212 = local write "Right Drive Zero"(w296) -> ()
          }
        }
      }
    }
  }
  n213 = Index Array(array=w42) -> (element=w40:refnum<vi>)  [unwired: 1 in]
  n214 = while {
    tunnel: w40 -> [w300]
    i -> [w303]
    stop <- FALSE stop-if-true
    n215 = Wait (ms)(milliseconds to wait=u32 100) -> ()  [unwired: 1 out]
    n216 = case shown="\"Playback\"" "Rec Mode" {
      tunnel: w303 -> [_ _ w318]
      tunnel: [u32 2829099 ("Base Color") u32 11141120 ("Target Color") w307] -> w299
      frame "Stop", Default {
        # "Reset the color, extra updates don't cost much"
      }
      frame "Record" {
      }
      frame "Playback" {
        # "Playback"
        n217 = Quotient & Remainder(x=w318, y=u32 50 ("milliseconds to wait")) -> (x-y*floor(x/y)=w314:u32)  [unwired: 1 out]
        n218 = Divide(x=w314, y=u32 50 ("milliseconds to wait")) -> (x/y=w311:dbl)
        n219 = Multiply(x=6.283185307179586, y=w311) -> (x*y=w316:dbl)
        n220 = Sine(x=w316) -> (sin(x)=w315:dbl)
        n221 = Absolute Value(x=w315) -> (abs(x)=w308:dbl)
        n222 = call "Interpolate RGB Color.vi"("Proportion"=w308, "Target Color"=u32 30976, "Base Color"=u32 2829099) -> ("Result Color"=w307:u32)  [unwired: 8 in]
      }
    }
    n223 = property class="Pane"(reference=w300, "PaneColor"=w299) -> ()  [unwired: 1 in, 2 out]
  }
  n224 = local write "Dashboard Tab"(T2."Auto" ("Dashboard Tab")) -> ()
  n225 = while {
    tunnel: u16 1741 ("timeout ms (25000)") -> [w320]
    stop <- FALSE stop-if-true
    n226 = TCP Create Listener(10:w320) -> (0:w319:errorcluster, 3:w321:refnum<k5>)  [unwired: 4 in, 1 out]
    n227 = case shown="No Error" w319 {
      selector: w319 -> [w323 _]
      tunnel: w321 -> [w324 _]
      frame No Error {
        n228 = while {
          tunnel: w324 -> [w327]
          tunnel: w323 -> [w326]
          stop <- FALSE stop-if-true
          n229 = TCP Wait On Listener(8:w326, 11:w327) -> (0:w328:errorcluster, 4:w329:refnum<k5>)  [unwired: 2 in, 3 out]
          n230 = local write "TCP"(w329) -> ()
          n231 = case shown="No Error" w328 {
            frame No Error {
            }
            frame Error {
              n232 = Wait (ms)(milliseconds to wait=u32 1000) -> ()  [unwired: 1 out]
            }
          }
        }
      }
      frame Error {
        n233 = Wait (ms)(milliseconds to wait=u32 1000) -> ()  [unwired: 1 out]
      }
    }
  }
  n234 = global write "WPI_DashboardLogging Global.vi" "Recording"(w35) -> ()
  n235 = local write "Rec Mode"(w35) -> ()
